vi "Send Data Loop.vi"(10 "connection ID":refnum<k5>, 11 "队列输入":refnum<queue>) -> ()   [LabVIEW 2020, in "TCP Communication.lvlib"]
uses:
  TCP Communication.lvlib
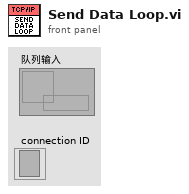
[diagram p1: front panel]
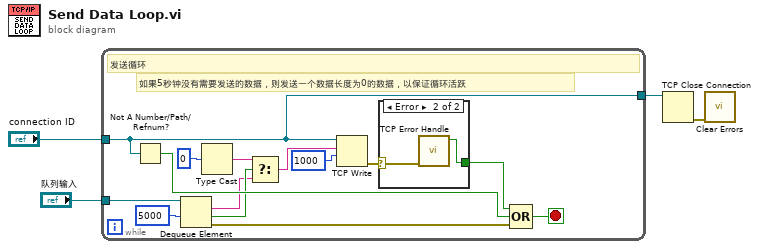
[diagram p0: block diagram]
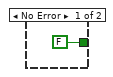
[diagram p2: hidden frame]
diagram:
  n1 = while {
    tunnel: "队列输入" -> [w18]
    tunnel: "connection ID" -> [w12]
    tunnel: [w12] -> w4
    stop <- w14 stop-if-true
    # "如果5秒钟没有需要发送的数据，则发送一个数据长度为0的数据，以保证循环活跃"
    # "发送循环"
    n2 = Not A Number/Path/Refnum?(number/path/refnum=w12) -> (NaN/Path/Refnum?=w13:bool)
    n3 = Dequeue Element(queue=w18, timeout in ms (-1)=5000 ("超时毫秒(-1)")) -> (element=w8:string, timed out?=w9:bool, error out=w11:errorcluster)  [unwired: 1 in, 1 out]
    n4 = Type Cast(x=0) -> (*(type *) &x=w5:string)  [unwired: 1 in]
    n5 = Select(t=w5, s=w9, f=w8) -> (s? t:f=w7:string)
    n6 = TCP Write(connection ID=w12, data in=w7, 9:1000 ("超时毫秒(25000)")) -> (error out=w16:errorcluster)  [unwired: 1 in, 2 out]
    n7 = case shown="Error" w16 {
      selector: w16 -> [_ w21]
      tunnel: [FALSE ("Stop?") w20] -> w15
      frame No Error {
      }
      frame Error {
        n8 = call "TCP Error Handle.vi"("错误输入（无错误）"=w21) -> ("Stop?"=w20:bool)  [unwired: 9 in, 1 out]
      }
    }
    n9 = Compound Arithmetic op=OR ("复合运算")(w15, w13, w11) -> (w14:bool)
  }
  n10 = TCP Close Connection(connection ID=w4) -> (error out=w3:errorcluster)  [unwired: 2 in, 1 out]
  n11 = call <vilib>:"Clear Errors.vi"("error in (no error)"=w3) -> ()  [unwired: 5 in, 2 out]
